vi "Pulse_Sequence.vi"() -> ()   [LabVIEW 2025]
doc: "This example demonstrates how to generate synchronized waveforms with any number of SMC-based PXI waveform generators in the same chassis or any number of SMC-based PCI waveform generators sharing a common RTSI bus. The waveform generators continuously generate synchronized square waves. Immediate trigger is used to start generation on all modules.\n\nAssumptions: \n\nFor PXI: Modules must be in one PXI chassis, because the PXI backplane is used for synchronization and trigger distribution. Ensure that the PXI chassis has been properly identified in MAX.\n\nFor PCI: Modules must be in one PCI computer, and connected with a RTSI bus because the RTSI bus is used for synchronization and trigger distribution. Ensure that MAX indicates that the cable was created and that synchronized instruments are connected to it."
uses:
  <instrlib>/niFgen/niFgen.llb/niFgen_ctl Trigger SW - TrigName Values (Ring).ctl
  <instrlib>/niFgen/niFgen.llb/niFgen_ctl Exported Signal Desination Values (ComboBox).ctl
  <instrlib>/niFgen/niFgen.llb/niFgen_ctl Exported Signal Name Values (Ring).ctl
  <instrlib>/niFgen/niFgen.llb/niFgen Trigger Mode.ctl
  <instrlib>/niFgen/niFgen.llb/niFgen Create Waveform (DBL).vi
  <vilib>/Analysis/NI_AALBase.lvlib
panel:
  in  "Sample Rate 2":dbl=50000000.0 format="%.2p"
  in  "width 2":i32=2000
  in  "delay 2":i32=1
  in  "delay":i32
  in  "width":i32=10000000
  in  "Resource Name 2":refnum<k15>="Dev2" caption="T set"
  in  "stop":bool
  in  "Resource Name":refnum<k15>="Dev3" caption="AOM"
  in  "Pulse Width (ns)":i32[](array[numeric])=[300, 100, 5]
  in  "Pulse Delay (ns)":i32[](array[numeric])=[1800, 100, 200]
  in  "Sample Rate":dbl=100000000.0 format="%.2p"
  in  "FGEN Resource Names":refnum<k15>[](array[refnum])=["Dev1"] caption="detector"
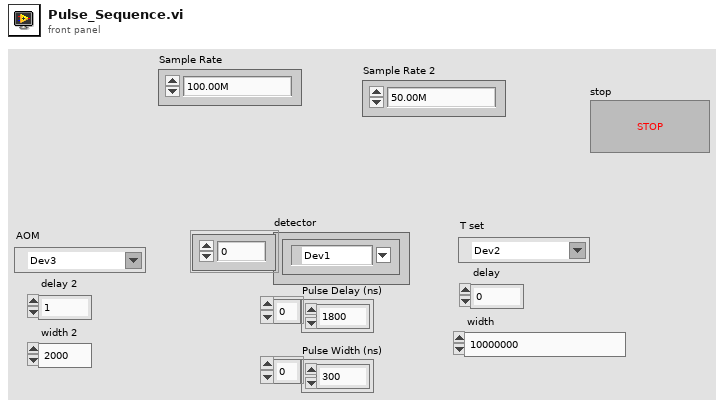
[diagram p1: front panel]
types:
  T1 = typedef "niFgen_ctl Trigger SW - TrigName Values (Ring).ctl" = i32
  T2 = typedef "niFgen Trigger Mode.ctl" = i32
  T3 = typedef "niFgen_ctl Exported Signal Name Values (Ring).ctl" = u16
  T4 = typedef "niFgen_ctl Exported Signal Desination Values (ComboBox).ctl" = string
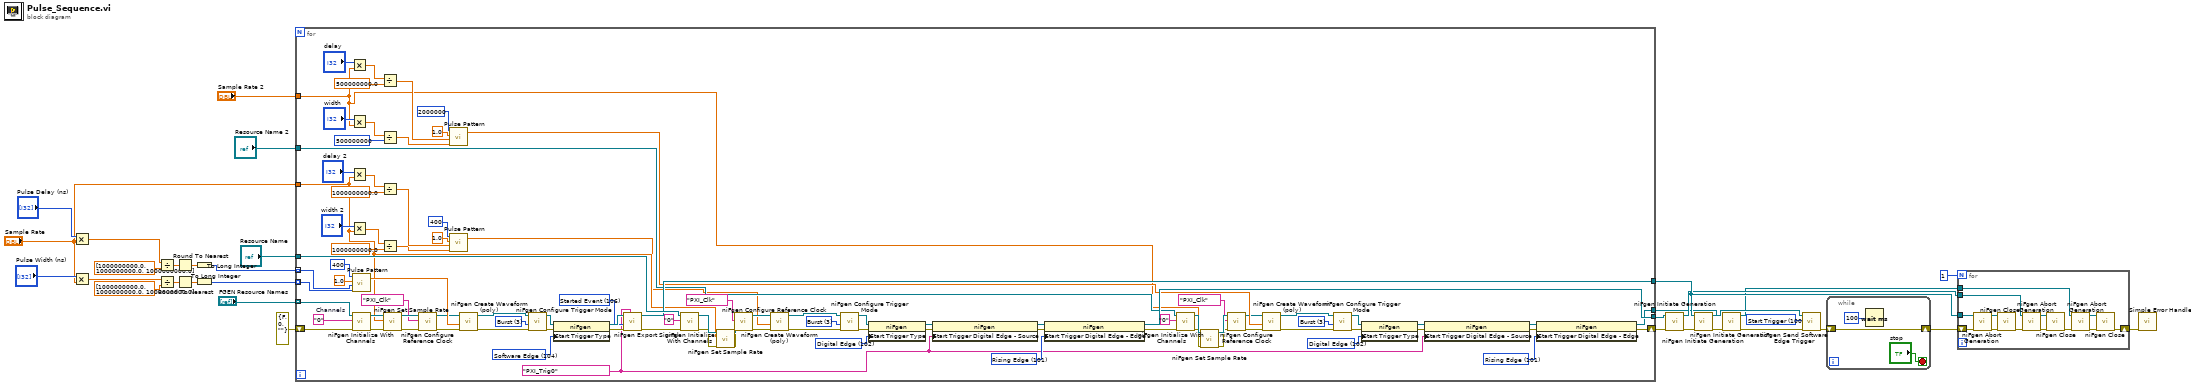
[diagram p0: block diagram]
diagram:
  w9 = T1 1004 items=["Start Trigger"=1004, "Script Trigger"=103] ("Trigger (Start Trigger)")
  n1 = Multiply(x="Pulse Delay (ns)", y="Sample Rate") -> (x*y=w31:dbl[])
  n2 = Multiply(x="Pulse Width (ns)", y="Sample Rate") -> (x*y=w23:dbl[])
  n3 = Divide(x=w31, y=dbl[] [1000000000.0, 1000000000.0, 1000000000.0]) -> (x/y=w29:dbl[])
  n4 = Divide(x=w23, y=dbl[] [1000000000.0, 1000000000.0, 1000000000.0]) -> (x/y=w21:dbl[])
  n5 = Round To Nearest(number=w29) -> (nearest integer value=w28:dbl[])
  n6 = Round To Nearest(number=w21) -> (nearest integer value=w20:dbl[])
  n7 = To Long Integer(number=w28) -> (32bit integer=w27:i32[])
  n8 = To Long Integer(number=w20) -> (32bit integer=w19:i32[])
  n9 = for {
    tunnel: "FGEN Resource Names" -> [w128] mode=indexing
    tunnel: [w83] -> w12
    shift-right: [w56] -> w15
    shift-left: errorcluster {"status"=FALSE, "code"=0, "source"=""} ("error") -> [w127]
    tunnel: "Sample Rate" -> [w42]
    tunnel: w27 -> [w120] mode=indexing
    tunnel: w19 -> [w119] mode=indexing
    tunnel: "Resource Name" -> [w118]
    tunnel: [w82] -> w14
    tunnel: "Resource Name 2" -> [w59]
    tunnel: [w55] -> w5
    tunnel: "Sample Rate 2" -> [w34]
    w61 = 101 items=["Rising Edge"=101, "Falling Edge"=102] ("Triggers:Start:Digital Edge:Edge")
    w70 = T2 3 items=["Single", "Continuous", "Stepped", "Burst"] ("Trigger Mode (default: 1=continuous)")
    w71 = 102 items=["None"=101, "Digital Edge"=102, "Software Edge"=104, "P2P Endpoint Fullness"=106] ("Triggers:Start:Trigger Type")
    w85 = 101 items=["Rising Edge"=101, "Falling Edge"=102] ("Triggers:Start:Digital Edge:Edge")
    w94 = T2 3 items=["Single", "Continuous", "Stepped", "Burst"] ("Trigger Mode (default: 1=continuous)")
    w95 = 102 items=["None"=101, "Digital Edge"=102, "Software Edge"=104, "P2P Endpoint Fullness"=106] ("Triggers:Start:Trigger Type")
    w96 = T3 106 items=["Sample Clock"=101, "Sample Clock Timebase"=1006, "Reference Clock"=102, "Onboard Reference Clock"=1019, "Start Trigger"=1004, "Script Trigger"=103, "Marker Event"=1001, "Data Marker Event"=108, "Ready For Start Event"=105, "Started Event"=106, "Done Event"=107, "Synchronization Pulse"=1007, "Sync Out"=1002] ("Signal")
    w99 = 104 items=["None"=101, "Digital Edge"=102, "Software Edge"=104, "P2P Endpoint Fullness"=106] ("Triggers:Start:Trigger Type")
    w60 = T4 "PXI_Trig0" ("Output Terminal (do not export)")
    w102 = T2 3 items=["Single", "Continuous", "Stepped", "Burst"] ("Trigger Mode (default: 1=continuous)")
    w124 = "0"  # Channels
    n10 = Multiply(x="delay", y=w34) -> (x*y=w49:dbl)
    n11 = Multiply(x="width", y=w34) -> (x*y=w51:dbl)
    n12 = Multiply(x="delay 2", y=w42) -> (x*y=w41:dbl)
    n13 = Multiply(x="width 2", y=w42) -> (x*y=w45:dbl)
    n14 = call <vilib>:"Pulse Pattern.vi"("width"=w119, "delay"=w120, "amplitude"=1.0, "samples"=400) -> ("Pulse Pattern"=w121:dbl[])  [unwired: 1 out]
    n15 = call <instrlib>:"niFgen Initialize With Channels.vi"("error in (no error)"=w127, "Channel Name"=w124, "Resource Name"=w128) -> ("error out"=w126:errorcluster, "Instrument Handle Out"=w125:refnum<k15>)  [unwired: 7 in]
    n16 = Divide(x=w49, y=500000000.0) -> (x/y=w47:dbl)
    n17 = Divide(x=w51, y=500000000) -> (x/y=w53:dbl)
    n18 = Divide(x=w41, y=1000000000.0) -> (x/y=w39:dbl)
    n19 = Divide(x=w45, y=1000000000.0) -> (x/y=w38:dbl)
    n20 = call <instrlib>:"niFgen Set Sample Rate.vi"("error in (no error)"=w126, "Sample Rate (Samp/s)"=w42, "Instrument Handle"=w125) -> ("error out"=w114:errorcluster, "Instrument Handle Out"=w115:refnum<k15>)  [unwired: 7 in]
    n21 = call <instrlib>:"niFgen Configure Reference Clock.vi"("error in (no error)"=w114, "Source"="PXI_Clk", "Instrument Handle"=w115) -> ("error out"=w113:errorcluster, "Instrument Handle Out"=w112:refnum<k15>)  [unwired: 7 in]
    n22 = call <vilib>:"Pulse Pattern.vi"("width"=w53, "delay"=w47, "amplitude"=1.0, "samples"=2000000) -> ("Pulse Pattern"=w79:dbl[])  [unwired: 1 out]
    n23 = call <vilib>:"Pulse Pattern.vi"("width"=w38, "delay"=w39, "amplitude"=1.0, "samples"=400) -> ("Pulse Pattern"=w35:dbl[])  [unwired: 1 out]
    n24 = call-poly <instrlib>:"niFgen Create Waveform (poly).vi"("error in (no error)"=w113, "Waveform Data Array"=w121, "Instrument Handle"=w112) -> ("error out"=w103:errorcluster, "Instrument Handle Out"=w104:refnum<k15>)  [unwired: 6 in, 1 out]
    n25 = call <instrlib>:"niFgen Configure Trigger Mode.vi"("error in (no error)"=w103, "Trigger Mode (default: 1=continuous)"=w102, "Instrument Handle"=w104) -> ("error out"=w100:errorcluster, "Instrument Handle Out"=w101:refnum<k15>)  [unwired: 7 in]
    n26 = property class="niFgen"(reference=w101, error in=w100, "Start Trigger Type"=w99) -> (reference out=w98:refnum<k15>, error out=w97:errorcluster)
    n27 = call <instrlib>:"niFgen Export Signal.vi"("Output Terminal (do not export)"=w60, "error in (no error)"=w97, "Signal"=w96, "Instrument Handle"=w98) -> ("error out"=w84:errorcluster, "Instrument Handle Out"=w83:refnum<k15>)  [unwired: 6 in]
    n28 = call <instrlib>:"niFgen Initialize With Channels.vi"("error in (no error)"=w84, "Channel Name"="0", "Resource Name"=w118) -> ("error out"=w107:errorcluster, "Instrument Handle Out"=w117:refnum<k15>)  [unwired: 7 in]
    n29 = call <instrlib>:"niFgen Set Sample Rate.vi"("error in (no error)"=w107, "Sample Rate (Samp/s)"=w42, "Instrument Handle"=w117) -> ("error out"=w106:errorcluster, "Instrument Handle Out"=w111:refnum<k15>)  [unwired: 7 in]
    n30 = call <instrlib>:"niFgen Configure Reference Clock.vi"("error in (no error)"=w106, "Source"="PXI_Clk", "Instrument Handle"=w111) -> ("error out"=w105:errorcluster, "Instrument Handle Out"=w108:refnum<k15>)  [unwired: 7 in]
    n31 = call-poly <instrlib>:"niFgen Create Waveform (poly).vi"("error in (no error)"=w105, "Waveform Data Array"=w35, "Instrument Handle"=w108) -> ("error out"=w92:errorcluster, "Instrument Handle Out"=w93:refnum<k15>)  [unwired: 6 in, 1 out]
    n32 = call <instrlib>:"niFgen Configure Trigger Mode.vi"("error in (no error)"=w92, "Trigger Mode (default: 1=continuous)"=w94, "Instrument Handle"=w93) -> ("error out"=w90:errorcluster, "Instrument Handle Out"=w91:refnum<k15>)  [unwired: 7 in]
    n33 = property class="niFgen"(reference=w91, error in=w90, "Start Trigger Type"=w95) -> (reference out=w89:refnum<k15>, error out=w88:errorcluster)
    n34 = property class="niFgen"(reference=w89, error in=w88, "Start Trigger Digital Edge - Source"=w60) -> (reference out=w87:refnum<k15>, error out=w86:errorcluster)
    n35 = property class="niFgen"(reference=w87, error in=w86, "Start Trigger Digital Edge - Edge"=w85) -> (reference out=w82:refnum<k15>, error out=w57:errorcluster)
    n36 = call <instrlib>:"niFgen Initialize With Channels.vi"("error in (no error)"=w57, "Channel Name"="0", "Resource Name"=w59) -> ("error out"=w74:errorcluster, "Instrument Handle Out"=w81:refnum<k15>)  [unwired: 7 in]
    n37 = call <instrlib>:"niFgen Set Sample Rate.vi"("error in (no error)"=w74, "Sample Rate (Samp/s)"=w34, "Instrument Handle"=w81) -> ("error out"=w73:errorcluster, "Instrument Handle Out"=w77:refnum<k15>)  [unwired: 7 in]
    n38 = call <instrlib>:"niFgen Configure Reference Clock.vi"("error in (no error)"=w73, "Source"="PXI_Clk", "Instrument Handle"=w77) -> ("error out"=w72:errorcluster, "Instrument Handle Out"=w75:refnum<k15>)  [unwired: 7 in]
    n39 = call-poly <instrlib>:"niFgen Create Waveform (poly).vi"("error in (no error)"=w72, "Waveform Data Array"=w79, "Instrument Handle"=w75) -> ("error out"=w68:errorcluster, "Instrument Handle Out"=w69:refnum<k15>)  [unwired: 6 in, 1 out]
    n40 = call <instrlib>:"niFgen Configure Trigger Mode.vi"("error in (no error)"=w68, "Trigger Mode (default: 1=continuous)"=w70, "Instrument Handle"=w69) -> ("error out"=w66:errorcluster, "Instrument Handle Out"=w67:refnum<k15>)  [unwired: 7 in]
    n41 = property class="niFgen"(reference=w67, error in=w66, "Start Trigger Type"=w71) -> (reference out=w65:refnum<k15>, error out=w64:errorcluster)
    n42 = property class="niFgen"(reference=w65, error in=w64, "Start Trigger Digital Edge - Source"=w60) -> (reference out=w63:refnum<k15>, error out=w62:errorcluster)
    n43 = property class="niFgen"(reference=w63, error in=w62, "Start Trigger Digital Edge - Edge"=w61) -> (reference out=w55:refnum<k15>, error out=w56:errorcluster)
  }
  n44 = call <instrlib>:"niFgen Initiate Generation.vi"("error in (no error)"=w15, "Instrument Handle"=w14) -> ("error out"=w13:errorcluster, "Instrument Handle Out"=w11:refnum<k15>)  [unwired: 8 in]
  n45 = call <instrlib>:"niFgen Initiate Generation.vi"("error in (no error)"=w13, "Instrument Handle"=w12) -> ("error out"=w4:errorcluster, "Instrument Handle Out"=w10:refnum<k15>)  [unwired: 8 in]
  n46 = call <instrlib>:"niFgen Initiate Generation.vi"("error in (no error)"=w4, "Instrument Handle"=w5) -> ("error out"=w3:errorcluster, "Instrument Handle Out"=w2:refnum<k15>)  [unwired: 8 in]
  n47 = call <instrlib>:"niFgen Send Software Edge Trigger.vi"("error in (no error)"=w3, "Trigger (Start Trigger)"=w9, "Instrument Handle"=w10) -> ("error out"=w8:errorcluster)  [unwired: 7 in, 1 out]
  n48 = while {
    shift-right: [w129] -> w7
    shift-left: w8 -> [w129]
    stop <- "stop" stop-if-true
    n49 = Wait (ms)(milliseconds to wait=u32 100) -> ()  [unwired: 1 out]
  }
  n50 = for {
    N: 1 -> [_]
    tunnel: w12 -> [w143]
    shift-right: [w132] -> w17
    shift-left: w7 -> [w140]
    tunnel: w11 -> [w142]
    tunnel: w2 -> [w134]
    n51 = call <instrlib>:"niFgen Abort Generation.vi"("error in (no error)"=w140, "Instrument Handle"=w143) -> ("error out"=w139:errorcluster, "Instrument Handle Out"=w144:refnum<k15>)  [unwired: 8 in]
    n52 = call <instrlib>:"niFgen Close.vi"("error in (no error)"=w139, "Instrument Handle"=w144) -> ("error out"=w138:errorcluster)  [unwired: 9 in]
    n53 = call <instrlib>:"niFgen Abort Generation.vi"("error in (no error)"=w138, "Instrument Handle"=w142) -> ("error out"=w137:errorcluster, "Instrument Handle Out"=w141:refnum<k15>)  [unwired: 8 in]
    n54 = call <instrlib>:"niFgen Close.vi"("error in (no error)"=w137, "Instrument Handle"=w141) -> ("error out"=w136:errorcluster)  [unwired: 9 in]
    n55 = call <instrlib>:"niFgen Abort Generation.vi"("error in (no error)"=w136, "Instrument Handle"=w134) -> ("error out"=w135:errorcluster, "Instrument Handle Out"=w133:refnum<k15>)  [unwired: 8 in]
    n56 = call <instrlib>:"niFgen Close.vi"("error in (no error)"=w135, "Instrument Handle"=w133) -> ("error out"=w132:errorcluster)  [unwired: 9 in]
  }
  n57 = call <vilib>:"Simple Error Handler.vi"("error in (no error)"=w17) -> ()  [unwired: 4 in, 5 out]
